vi "Test MQTT-3.8.4-3.vi"(8 "error in (no error)":errorcluster, 11 "Connection Config":refnum<class "Connection.lvclass">) -> (0 "error out":errorcluster, 3 "Connection Config dup":refnum<class "Connection.lvclass">)   [LabVIEW 2013]
uses:
  <vilib>/LabVIEW Open Source Project/MQTT Connection/MQTT_Connection/Connection/Connection.lvclass
  <vilib>/LabVIEW Open Source Project/MQTT Control Packets/Control Packets/SUBSCRIBE/Topic Subscription -- cluster.ctl
  <vilib>/LabVIEW Open Source Project/MQTT Control Packets/Control Packets/ControlPacket/QualityOfService -- enum.ctl
  <vilib>/addons/_JKI Toolkits/Caraya/classes/Test/Test.lvclass
  <vilib>/LabVIEW Open Source Project/MQTT Client/Client class/Client.lvclass
  <vilib>/LabVIEW Open Source Project/MQTT Control Packets/Control Packets/SUBSCRIBE/SUBSCRIBE.lvclass
  <vilib>/addons/_JKI Toolkits/Caraya/classes/Assert/Assert.lvclass
  <vilib>/LabVIEW Open Source Project/MQTT Connection/MQTT_Base/Base Class/MQTT_Base.lvclass
  <vilib>/LabVIEW Open Source Project/MQTT Control Packets/Control Packets/ControlPacket/ControlPacket.lvclass
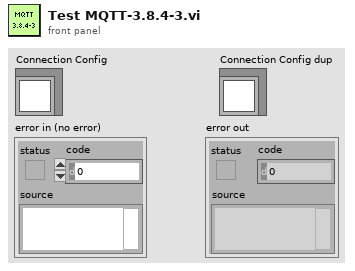
[diagram p1: front panel]
types:
  T1 = typedef "MQTT_Control_Packets.lvlib/SUBSCRIBE.lvclass/Topic Subscription -- cluster.ctl" = cluster{"Topic Filter":string, "QoS":T2}
  T2 = typedef "MQTT_Control_Packets.lvlib/ControlPacket.lvclass/QualityOfService -- enum.ctl" = enum16{"0 (At Most Once)", "1 (At Least Once)", "2 (Exactly Once)"}
  T3 = typedef "MQTT_Control_Packets.lvlib/SUBACK.lvclass/Subscription Success Code.ctl" = cluster{"Subscription Failure":bool, "QoS":T2}
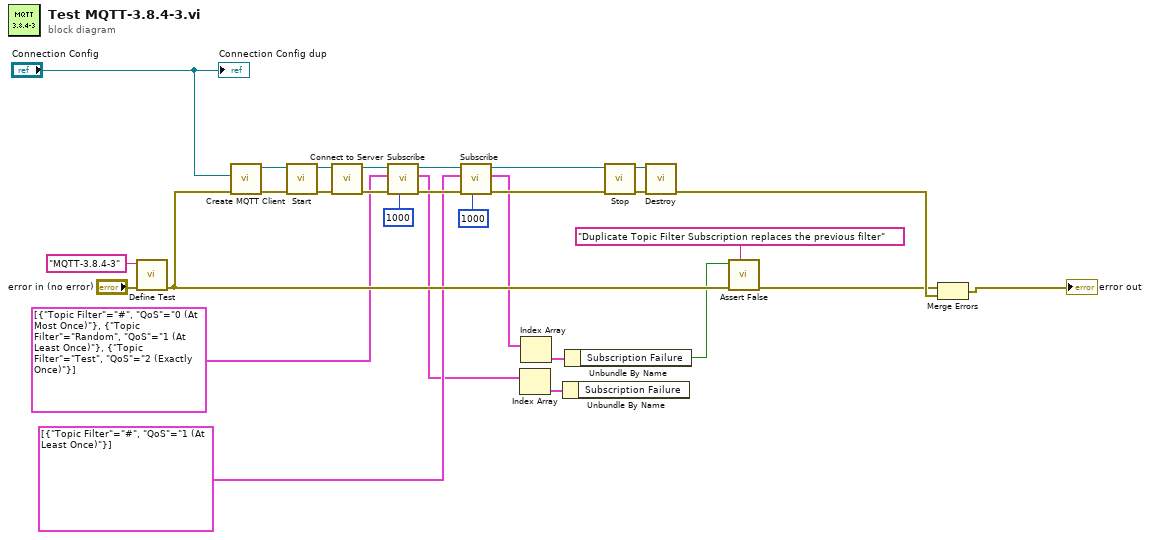
[diagram p0: block diagram]
diagram:
  n1 = call <vilib>:"Define Test.vi"("error in (no error)"="error in (no error)", "Label (VI Title)"="MQTT-3.8.4-3") -> ("error out"=w16:errorcluster)  [unwired: 9 in]
  n2 = call <vilib>:"Create MQTT Client.vi"("error in (no error)"=w16, "Connection Configuration"="Connection Config") -> ("error out"=w18:errorcluster, "Client out"=w19:refnum<class "Client.lvclass">)  [unwired: 8 in]
  n3 = call <vilib>:"Start.vi"("error in (no error)"=w18, "MQTT_Base in"=w19) -> ("error out"=w25:errorcluster, "MQTT_Base out"=w26:refnum<class "Client.lvclass">)  [unwired: 7 in, 1 out]
  n4 = call <vilib>:"Connect to Server.vi"("error in (no error)"=w25, "Client in"=w26) -> ("error out"=w21:errorcluster, "Client out"=w22:refnum<class "Client.lvclass">)  [unwired: 6 in, 2 out]
  n5 = call <vilib>:"Subscribe.vi"("timeout (1000 ms)"=1000, "error in (no error)"=w21, "Topic Subscriptions"=T1[] [{"Topic Filter"="#", "QoS"=enum."0 (At Most Once)"}, {"Topic Filter"="Random", "QoS"=enum."1 (At Least Once)"}, {"Topic Filter"="Test", "QoS"=enum."2 (Exactly Once)"}], "MQTT_Base in"=w22) -> ("error out"=w10:errorcluster, "Subscription Success"=w6:T3[], "MQTT_Base out"=w12:refnum<class "Client.lvclass">)  [unwired: 4 in, 1 out]
  n6 = call <vilib>:"Subscribe.vi"("timeout (1000 ms)"=1000, "error in (no error)"=w10, "Topic Subscriptions"=T1[] [{"Topic Filter"="#", "QoS"=enum."1 (At Least Once)"}], "MQTT_Base in"=w12) -> ("error out"=w9:errorcluster, "Subscription Success"=w5:T3[], "MQTT_Base out"=w11:refnum<class "Client.lvclass">)  [unwired: 4 in, 1 out]
  n7 = Index Array(array=w6) -> (element=w3:T3)  [unwired: 1 in]
  n8 = Index Array(array=w5) -> (element=w4:T3)  [unwired: 1 in]
  n9 = Unbundle By Name(w3) -> ()  [unwired: 1 out]
  n10 = Unbundle By Name(w4) -> ("Subscription Failure"=w2:bool)
  n11 = call <vilib>:"Stop.vi"("error in (no error)"=w9, "MQTT_Base in"=w11) -> ("error out"=w23:errorcluster, "MQTT_Base out"=w24:refnum<class "Client.lvclass">)  [unwired: 7 in, 1 out]
  n12 = call <vilib>:"Destroy.vi"("error in (no error)"=w23, "MQTT_Base in"=w24) -> ("error out"=w15:errorcluster)  [unwired: 8 in, 1 out]
  n13 = call <vilib>:"Assert False.vi"("Label"="Duplicate Topic Filter Subscription replaces the previous filter", "error in (no error)"=w16, "False?"=w2) -> ("error out"=w14:errorcluster)  [unwired: 8 in]
  n14 = Merge Errors(w14, w15) -> (→"error out":errorcluster)
  "Connection Config dup" <- "Connection Config"
